vi "Load Replay Samples.vi"(8 "error in":errorcluster, 10 "Load From ProgramData":bool, 11 "Run ID":string) -> (0 "error out":errorcluster, 3 "ReplaySamples":T1[](array[typedef]))   [LabVIEW 2026, in "dependencies.lvlib"]
uses:
  KeyboardAndMouseDataAcquisition.ctl
  KeyType.ctl
  51ae6a63-6c69-4fc5-bd9a-224650780877.vi
  <vilib>/JDP Science/JSONtext/JSON text to Variant.vi
  <vilib>/JDP Science/JSONtext/LVClass Serializer/JSONtext LVClass Serializer.lvclass
  dependencies.lvlib
panel:
  out "error out 2":errorcluster
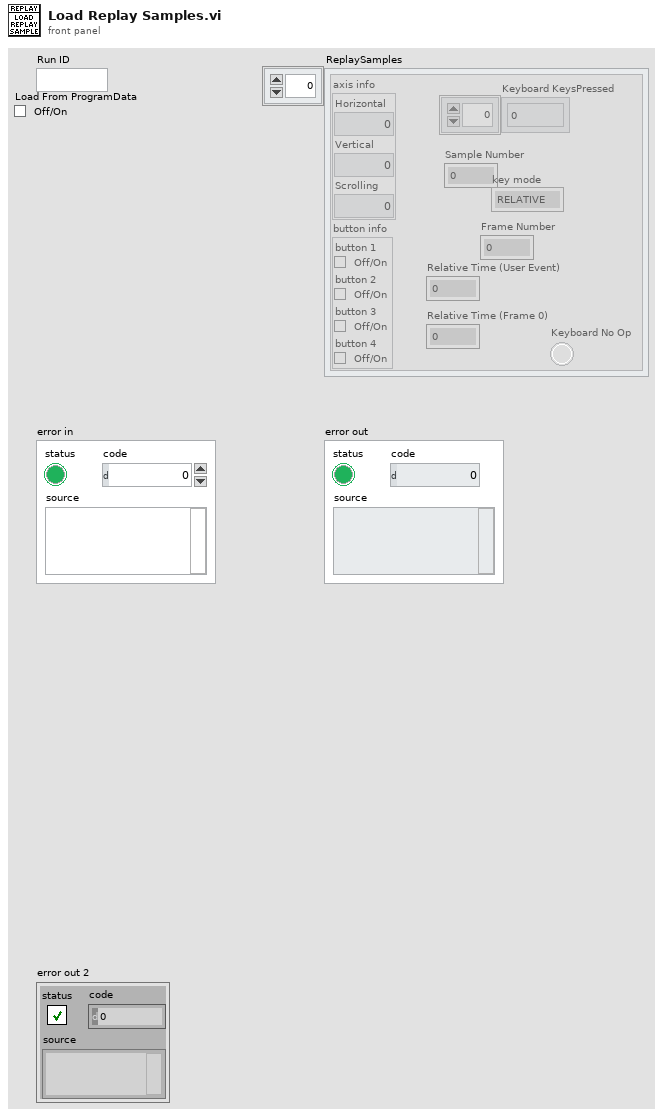
[diagram p1: front panel]
types:
  T1 = typedef "dependencies.lvlib/KeyboardAndMouseDataAcquisition.ctl" = cluster{"axis info":cluster{"Horizontal":i32, "Vertical":i32, "Scrolling":i32}, "button info":cluster{"button 1":bool, "button 2":bool, "button 3":bool, "button 4":bool}, "Relative Time (User Event)":dbl, "Sample Number":u32, "Relative Time (Frame 0)":dbl, "key mode":enum16{"RELATIVE", "ABSOLUTE"}, "Frame Number":u32, "Keyboard KeysPressed":T2[], "Keyboard No Op":bool}
  T2 = typedef "dependencies.lvlib/KeyType.ctl" = enum16{"0", "1", "2", "3", "4", "5", "6", "7", "8", "9", "A", "B", "C", "D", "E", "F", "G", "H", "I", "J", "K", "L", "M", "N", "O", "P", "Q", "R", "S", "T", "U", "V", "W", "X", "Y", "Z", "F1", "F2", "F3", "F4", "F5", "F6", "F7", "F8", "F9", "F10", "F11", "F12", "F13", "F14", "F15", "ADD", "BACK", "BACKSLASH", "CAPITAL", "COMMA", "DECIMAL", "DELETE", "DIVIDE", "DOWN", "END", "EQUALS", "ESCAPE", "GRAVE (`)", "HOME", "INSERT", "LBRACKET", "LCONTROL", "LEFT", "L ALT", "LSHIFT", "LWIN", "MINUS", "MULTIPLY", "NEXT", "NUMLOCK", "NUMPAD_0", "NUMPAD_1", "NUMPAD_2", "NUMPAD_3", "NUMPAD_4", "NUMPAD_5", "NUMPAD_6", "NUMPAD_7", "NUMPAD_8", "NUMPAD_9", "PAUSE", "PERIOD", "PRIOR (PG UP)", "RBRACKET", "RCONTROL", "RETURN", "RIGHT", "R ALT", "RSHIFT", "RWIN", "SCROLL", "SEMICOLON", "SLASH", "SPACE", "SUBTRACT", "TAB", "UP", "ENTER (num pad)", "' (quote)"}
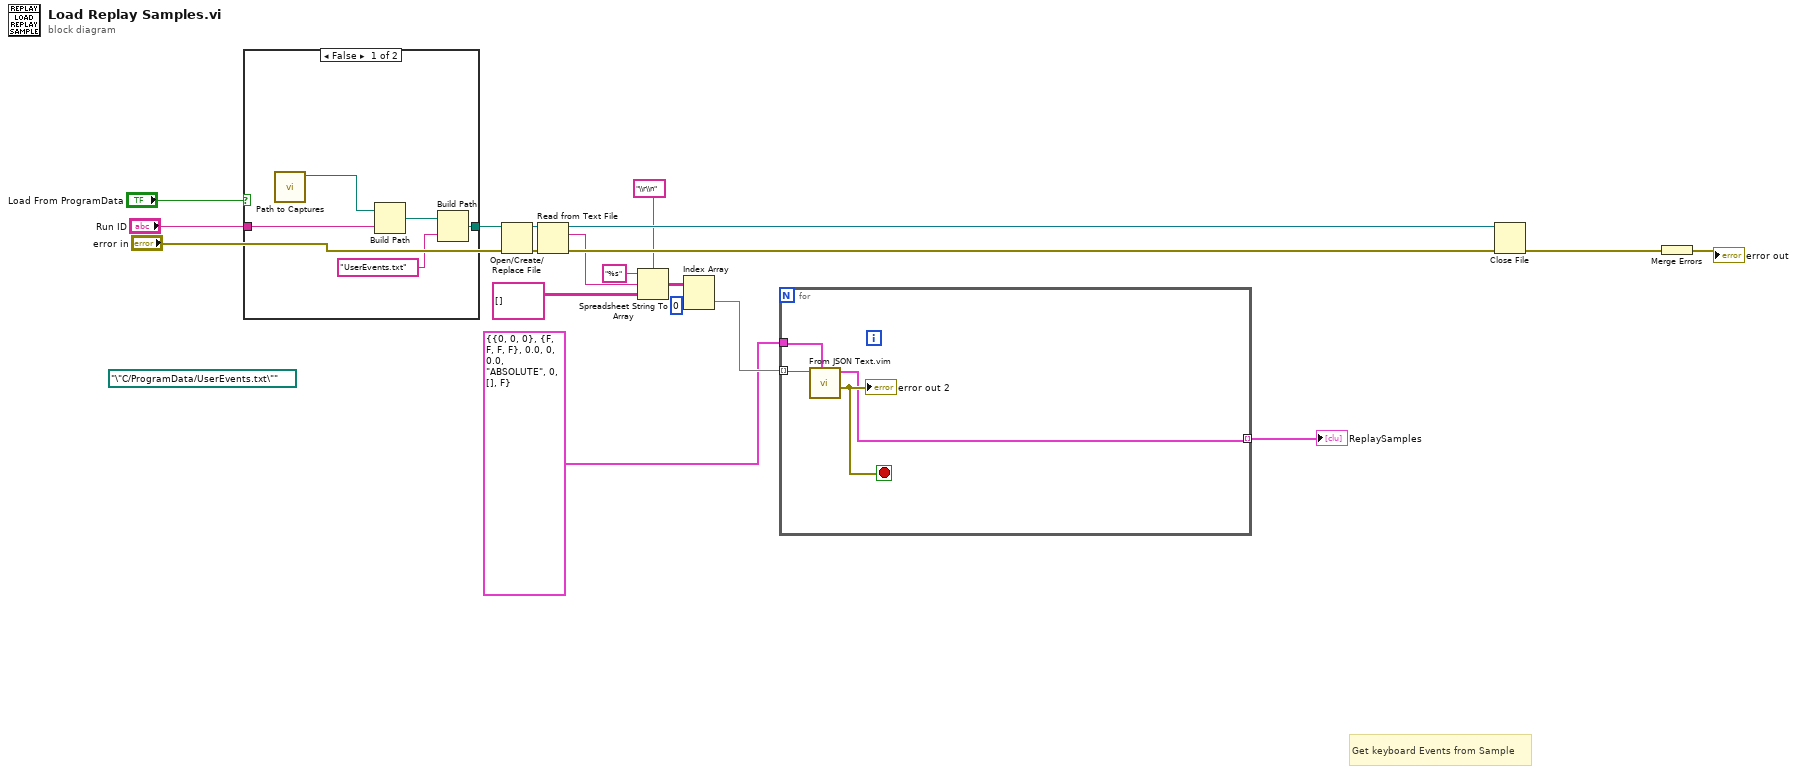
[diagram p0: block diagram]
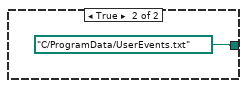
[diagram p2: hidden frame]
diagram:
  (unwired) path "/\"C/ProgramData/UserEvents.txt\"" ("appended path")
  # "Get keyboard Events from Sample"
  n1 = case shown="False" "Load From ProgramData" {
    tunnel: [w24 path "C:/ProgramData/UserEvents.txt" ("appended path")] -> w19
    tunnel: "Run ID" -> [w23 _]
    frame False {
      n2 = call "Path to Captures.vi"() -> ("Captures"=w22:path)  [unwired: 11 in]
      n3 = Build Path(base path=w22, name or relative path=w23) -> (appended path=w20:path)
      n4 = Build Path(base path=w20, name or relative path="UserEvents.txt" ("Run ID")) -> (appended path=w24:path)
    }
    frame True {
    }
  }
  n5 = Open/Create/Replace File(file path (use dialog)=w19, error in="error in") -> (refnum out=w16:refnum<file>, error out=w18:errorcluster)  [unwired: 4 in, 1 out]
  n6 = Read from Text File(file (use dialog)=w16, error in=w18) -> (refnum out=w15:refnum<file>, text=w13:string, error out=w17:errorcluster)  [unwired: 2 in, 1 out]
  n7 = Spreadsheet String To Array(delimiter (Tab)="\\r\\n", format string="%s", spreadsheet string=w13, array type (2D Dbl)=string[][] [] ("text")) -> (array=w10:string[][])
  n8 = Index Array(array=w10, index (col)=0 ("disabled index (col)")) -> (element=w4:string[])  [unwired: 1 in]
  n9 = for {
    tunnel: w4 -> [w29] mode=indexing
    tunnel: T1 {"axis info"={"Horizontal"=0, "Vertical"=0, "Scrolling"=0}, "button info"={"button 1"=FALSE, "button 2"=FALSE, "button 3"=FALSE, "button 4"=FALSE}, "Relative Time (User Event)"=0.0, "Sample Number"=0, "Relative Time (Frame 0)"=0.0, "key mode"=enum."ABSOLUTE", "Frame Number"=0, "Keyboard KeysPressed"=[], "Keyboard No Op"=FALSE} ("KeyboardAndMouseData") -> [w27]
    tunnel: [w26] -> w3 mode=indexing
    stop <- w28 stop-if-true
    n10 = call "From JSON Text.vim"("Data Type and Default Value"=w27, "JSON"=w29) -> ("error out"=w28:errorcluster, "Data out"=w26:T1)  [unwired: 8 in]
    "error out 2" <- w28
  }
  "ReplaySamples" <- w3
  n11 = Close File(refnum=w15, error in=w17) -> (error out=w6:errorcluster)  [unwired: 1 out]
  n12 = Merge Errors(w6) -> (→"error out":errorcluster)
